vi "Load User Prefs.vi"(8 "error in (no error)":errorcluster, 11 "Historian Charting Manager in":refnum<class "Historian Charting Manager.lvclass">) -> (0 "error out":errorcluster, 3 "Historian Charting Manager out":refnum<class "Historian Charting Manager.lvclass">)   [LabVIEW 2020, in "VolatusGUI.lvlib" / "Historian Charting Manager.lvclass"]
uses:
  Historian Charting Manager.lvclass
  Historian Charting Manager.lvclass/Historian Charting Manager.ctl
  lv-userprefs/User Prefs/Pref Group/Pref Group.lvclass
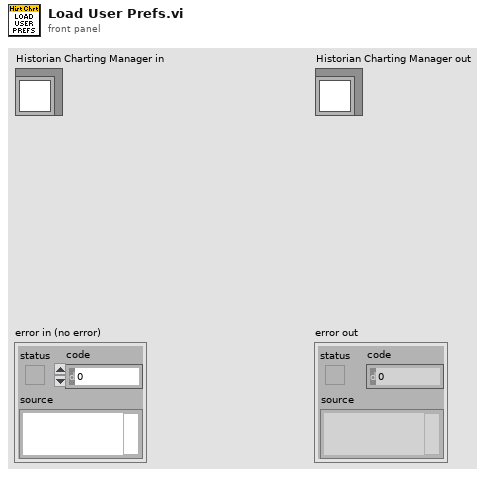
[diagram p1: front panel]
types:
  T1 = typedef "VolatusGUI.lvlib/Historian Charting Manager.lvclass/Plot Group Config.ctl" = cluster{"Name":string, "X-Axis Type":T2, "X-Axis Channel":string, "Plots":T3[], "Lock Now":bool, "Time":string, "Swap Axes":bool}
  T2 = typedef "VolatusGUI.lvlib/Historian Charting Manager.lvclass/X-Axis Type.ctl" = enum16{"Time", "Channel"}
  T3 = typedef "VolatusGUI.lvlib/Historian Charting Manager.lvclass/Plot Config.ctl" = cluster{"Channel":string, "Visible":bool, "Color":u32, "Scale":T4}
  T4 = typedef "VolatusGUI.lvlib/Historian Charting Manager.lvclass/Scale.ctl" = enum16{"Left", "Right"}
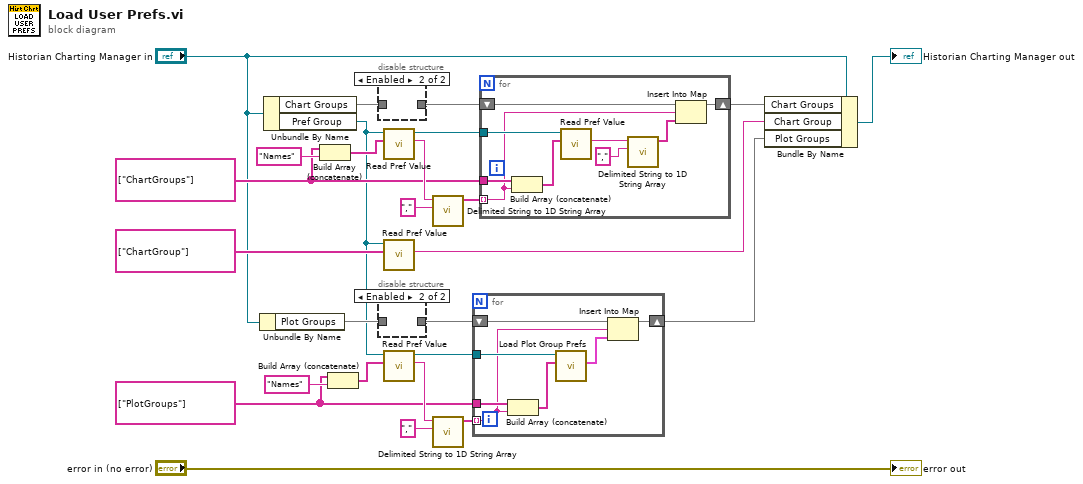
[diagram p0: block diagram]
diagram:
  w6 = string[] ["PlotGroups"] ("Pref Hierarchy")
  w16 = string[] ["ChartGroups"] ("Pref Hierarchy")
  n1 = Unbundle By Name("Historian Charting Manager in") -> ("Plot Groups"=w5:map{string, T1})
  n2 = Unbundle By Name("Historian Charting Manager in") -> ("Chart Groups"=w15:map{string, string[]}, "Pref Group"=w1:refnum<class "Pref Group.lvclass">)
  n3 = Build Array (concatenate)(w16, "Names") -> (w20:string[])
  n4 = Build Array (concatenate)(w6, "Names") -> (w17:string[])
  n5 = disable-structure shown="Enabled" {
    disable-tunnel: [w27 _] -> w14
    disable-tunnel: w15 -> [w27 _]
    frame Disabled {
    }
    frame Enabled {
    }
  }
  n6 = disable-structure shown="Enabled" {
    disable-tunnel: [w28 _] -> w4
    disable-tunnel: w5 -> [w28 _]
    frame Disabled {
    }
    frame Enabled {
    }
  }
  n7 = call "Read Pref Value.vi"("Pref Hierarchy"=w20, "Pref Group in"=w1) -> ("Value"=w24:string, "Pref Group out"=w21:refnum<class "Pref Group.lvclass">)  [unwired: 7 in, 1 out]
  n8 = call "Read Pref Value.vi"("Pref Hierarchy"=string[] ["ChartGroup"], "Pref Group in"=w1) -> ("Value"=w11:string)  [unwired: 7 in, 2 out]
  n9 = call "Read Pref Value.vi"("Pref Hierarchy"=w17, "Pref Group in"=w1) -> ("Value"=w9:string, "Pref Group out"=w7:refnum<class "Pref Group.lvclass">)  [unwired: 7 in, 1 out]
  n10 = call <vilib>:"Delimited String to 1D String Array.vi"("delimiter"=",", "delimited string"=w24) -> ("string array"=w22:string[])  [unwired: 9 in]
  n11 = call <vilib>:"Delimited String to 1D String Array.vi"("delimiter"=",", "delimited string"=w9) -> ("string array"=w8:string[])  [unwired: 9 in]
  n12 = for {
    tunnel: w8 -> [w30] mode=indexing
    tunnel: w7 -> [w34]
    tunnel: w6 -> [w35]
    shift-right: [w29] -> w3
    shift-left: w4 -> [w32]
    n13 = Build Array (concatenate)(w35, w30) -> (w33:string[])
    n14 = call "Load Plot Group Prefs.vi"("Hierarchy"=w33, "Pref Group in"=w34) -> ("Plot Group Config"=w31:T1)  [unwired: 9 in]
    n15 = Insert Into Map(map in=w32, key=w30, value=w31) -> (map out=w29:map{string, T1})  [unwired: 2 out]
  }
  n16 = for {
    tunnel: w22 -> [w40] mode=indexing
    tunnel: w21 -> [w43]
    tunnel: w16 -> [w44]
    shift-right: [w39] -> w13
    shift-left: w14 -> [w41]
    n17 = Build Array (concatenate)(w44, w40) -> (w42:string[])
    n18 = call "Read Pref Value.vi"("Pref Hierarchy"=w42, "Pref Group in"=w43) -> ("Value"=w37:string)  [unwired: 7 in, 2 out]
    n19 = call <vilib>:"Delimited String to 1D String Array.vi"("delimiter"=",", "delimited string"=w37) -> ("string array"=w36:string[])  [unwired: 9 in]
    n20 = Insert Into Map(map in=w41, key=w40, value=w36) -> (map out=w39:map{string, string[]})  [unwired: 2 out]
  }
  n21 = Bundle By Name(cluster="Historian Charting Manager in", "Chart Groups"=w13, "Chart Group"=w11, "Plot Groups"=w3) -> (→"Historian Charting Manager out":refnum<class "Historian Charting Manager.lvclass">)
  "error out" <- "error in (no error)"
